vi "Write Boolean Control Value.vi"(8 "error in (no error)":errorcluster, 10 "Boolean":bool, 11 "Boolean in":refnum<vi>) -> (0 "error out":errorcluster)   [LabVIEW 2021]
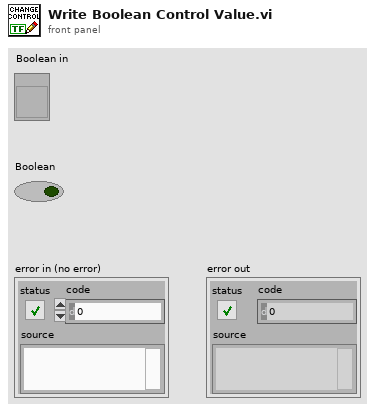
[diagram p1: front panel]
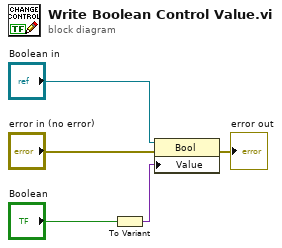
[diagram p0: block diagram]
diagram:
  n1 = To Variant(anything="Boolean") -> (Variant=w4:variant)
  n2 = property class="Bool"(reference="Boolean in", error in="error in (no error)", "Value"=w4) -> (error out=→"error out":errorcluster)  [unwired: 1 out]
